vi "GetCudaEnabledDeviceCount.vi"(8 "error in":errorcluster) -> (0 "error out":errorcluster, 3 "Count":i32)   [LabVIEW 2020, in "OpenLvVision_OpenCv.lvlib" / "Cuda.lvlib"]
doc: "Returns the number of installed CUDA-enabled devices."
uses:
  Cuda.lvlib
  OpenLvVision_OpenCv.lvlib
  Dlls/OlvOpenCvWrapper.dll
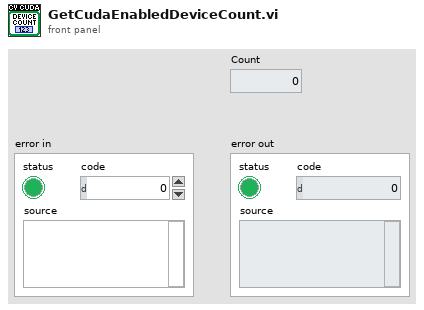
[diagram p1: front panel]
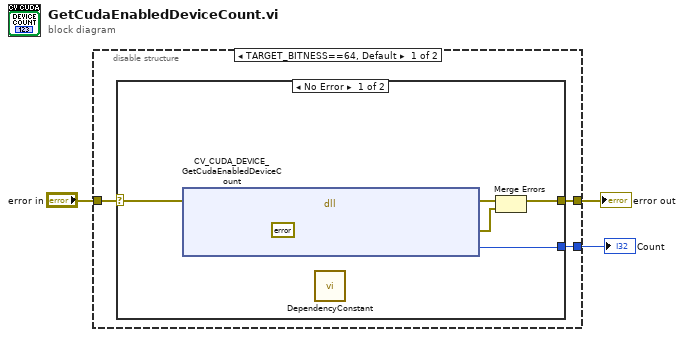
[diagram p0: block diagram]
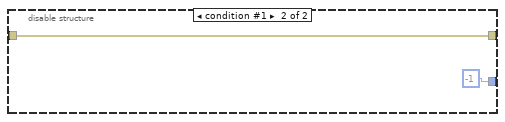
[diagram p3: hidden frame]
diagram:
  n1 = disable-structure shown="TARGET_BITNESS==64, Default" {
    disable-tunnel: "error in" -> [w5 w14]
    disable-tunnel: [w6 w14] -> w2
    disable-tunnel: [w4 -1 ("count")] -> w1
    frame condition #0 (active) {
      n2 = case shown="No Error" w5 {
        selector: w5 -> [w8 w13]
        tunnel: [w9 w13] -> w6
        tunnel: [w7 _] -> w4
        frame No Error {
          n3 = dll-call lib="C:/Users/lukas/Documents/OpenLvVision_OpenCv/SourceCode/LabView/OpenLvVision_OpenCv/Dlls/OlvOpenCvWrapper.dll" fn="CV_CUDA_DEVICE_GetCudaEnabledDeviceCount"(error in=w8, "Error"=errorcluster {"status"=FALSE, "code"=0, "source"=""} ("error out")) -> (error out=w12:errorcluster, "Error"=w11:errorcluster, "count"=w7:i32)  [unwired: 4 in, 1 out]
          n4 = call "DependencyConstant.vi"() -> ()  [unwired: 12 in]
          n5 = Merge Errors(w12, w11) -> (w9:errorcluster)
        }
        frame Error {
        }
      }
    }
    frame condition #1 {
    }
  }
  "error out" <- w2
  "Count" <- w1
